vi "nominal teststand convert results.vi"(10 "property bag":refnum<k7>, 11 "Sequence Context In":refnum<k7>) -> (1 "numerics":T1[](array[typedef]), 2 "strings":T2(array[cluster]), 3 "Report Text":string)   [LabVIEW 2020, in "nominal teststand model sequence support.lvlib"]
doc: "Theory of operation:\nFind all AdditionalResults\nGet Parent -> TS -> Start Time\nRecurse down AdditionalResults for data values\n\nParameters.MainSequenceResult->TS.StartTime\nseconds since start of engine for sequence\n\nParameters.MainSequenceResult->TS.SequenceCall.ResultList[0].TS.StartTime\nstep start time <- want this as timestamp for additional results\n\nresults we want\nParameters.MainSequenceResult->TS.SequenceCall.ResultList[0].AdditionalResults[\"result a1\"]"
uses:
  nominal teststand model sequence support.lvlib
  nominal numeric result collection.ctl
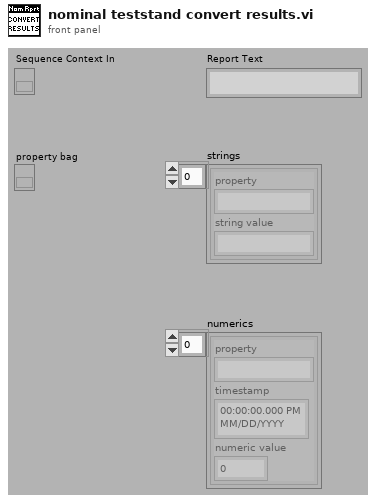
[diagram p1: front panel]
types:
  T1 = typedef "nominal teststand model sequence support.lvlib/nominal numeric result collection.ctl" = cluster{"property":string, "timestamp":timestamp, "numeric value":dbl}
  T2 = cluster{"property":string, "string value":string}[]
  T3 = cluster{timestamp, "strings":cluster{"property":string, "string value":string}[], "numerics":T1[], string}
  T4 = map{string, cluster{"possible timestamp":timestamp, "original property":T1}}
  T5 = map{string, cluster{"possible timestamp":timestamp, "original property":cluster{"property":string, "string value":string}}}
  T6 = cluster{"possible timestamp":timestamp, "original property":cluster{"property":string, "string value":string}}
  T7 = cluster{"possible timestamp":timestamp, "original property":T1}
  T8 = cluster{"property":string, "string value":string}
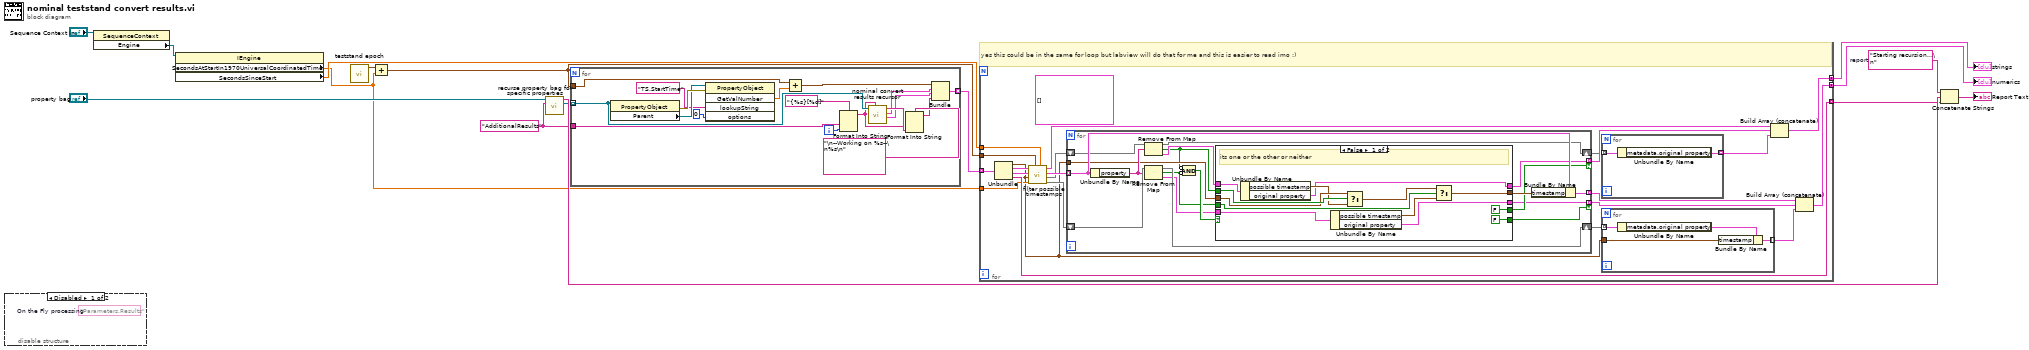
[diagram p0: block diagram]
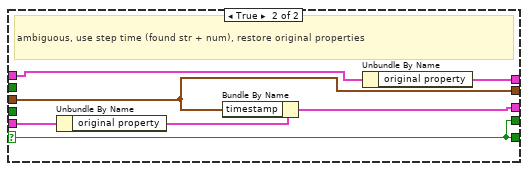
[diagram p2: hidden frame]
diagram:
  w8 = "AdditionalResults" ("search key (match pattern)")
  w15 = "Starting recursion...\n"  # report
  n1 = disable-structure shown="Disabled" {
    frame Disabled {
      (unwired) "Parameters.Results"  # On the Fly processing
    }
    frame Enabled {
    }
  }
  n2 = property class="SequenceContext"(reference="Sequence Context In") -> ("Engine"=w13:refnum<k7>)  [unwired: 1 in, 2 out]
  n3 = property class="IEngine"(reference=w13) -> ("SecondsAtStartIn1970UniversalCoordinatedTime"=w3:dbl, "SecondsSinceStart"=w4:dbl)  [unwired: 1 in, 2 out]
  n4 = call "teststand epoch.vi"() -> ("time stamp"=w12:timestamp)  [unwired: 11 in]
  n5 = Add(x=w12, y=w3) -> (x+y=w5:timestamp)
  n6 = call "recurse property bag for specific properties.vi"("search key (match pattern)"=w8, "property bag"="property bag") -> ("matching properties"=w9:refnum<k7>[], "Report Text"=w10:string)  [unwired: 8 in]
  n7 = for {
    tunnel: w9 -> [w28] mode=indexing
    tunnel: w5 -> [w29]
    tunnel: w8 -> [w24]
    tunnel: [w18] -> w7 mode=indexing
    i -> [w23]
    n8 = property class="PropertyObject"(reference=w28) -> (error out=w33:errorcluster, "Parent"=w32:refnum<k7>)  [unwired: 1 in, 1 out]
    n9 = invoke class="PropertyObject" method="GetValNumber"(reference=w32, error in=w33, "lookupString"="TS.StartTime" ("Lookup String"), "options"=0) -> ("GetValNumber"=w30:dbl)  [unwired: 1 in, 4 out]
    n10 = Add(x=w29, y=w30) -> (x+y=w21:timestamp)
    n11 = Format Into String(format string="{%s}[%d]", w24, w23) -> (resulting string=w22:string)  [unwired: 2 in, 1 out]
    n12 = call "nominal convert results recursor.vi"("hierarchy path"=w22, "property bag"=w28) -> ("numerics"=w19:T1[], "strings"=w20:T2, "Report Text"=w26:string)  [unwired: 7 in]
    n13 = Format Into String(format string="\n--Working on %s--\n%s\n", w22, w26) -> (resulting string=w17:string)  [unwired: 2 in, 1 out]
    n14 = Bundle(w21, "strings"=w20, "numerics"=w19, w17) -> (w18:T3)  [unwired: 1 in]
  }
  n15 = for {
    tunnel: w7 -> [w55] mode=indexing
    tunnel: [w54] -> w6 mode=indexing
    tunnel: w5 -> [w51]
    tunnel: w4 -> [w50]
    tunnel: w3 -> [w49]
    tunnel: [w47] -> w2 mode=concatenating
    tunnel: [w40] -> w1 mode=concatenating
    (unwired) T1[] [] ("numerics")
    # "yes this could be in the same for loop but labview will do that for me and this is easier to read imo :)"
    n16 = Unbundle(w55) -> (w35:timestamp, "strings"=w52:T2, "numerics"=w53:T1[], w54:string)
    n17 = call "filter possible timestamps.vi"("SecondsSinceStart"=w50, "engine start"=w51, "seconds at start"=w49, "step time"=w35, "numerics"=w53, "strings"=w52) -> ("possible timestamp numeric matches"=w44:T4, "possible timestamp string matches"=w45:T5, "remaining numerics"=w46:T1[], "remaining strings"=w48:T2)  [unwired: 2 in]
    n18 = for {
      tunnel: w46 -> [w78] mode=indexing
      tunnel: w35 -> [w68]
      tunnel: [w79] -> w43 mode=indexing
      shift-right: [w74] -> w39
      shift-left: w45 -> [w77]
      shift-right: [w73] -> w37
      shift-left: w44 -> [w76]
      tunnel: [w67] -> w41 mode=indexing if=w66
      tunnel: [w65] -> w42 mode=indexing if=w64
      n19 = Unbundle By Name(w78) -> ("property"=w75:string)
      n20 = Remove From Map(10:w75, 11:w77) -> (1:w70:T6, 2:w63:bool, 3:w74:T5)
      n21 = Remove From Map(10:w75, 11:w76) -> (1:w71:T7, 2:w62:bool, 3:w73:T4)
      n22 = Compound Arithmetic op=AND(invert w63, invert w62) -> (w72:bool)
      n23 = case shown="False" w72 {
        selector: w72 -> [_ w93]
        tunnel: w71 -> [w92 w97]
        tunnel: w70 -> [w91 w99]
        tunnel: [w84 w95] -> w69
        tunnel: w68 -> [w89 w95]
        tunnel: [w80 w98] -> w67
        tunnel: [FALSE w93] -> w66
        tunnel: [w81 w94] -> w65
        tunnel: [FALSE w93] -> w64
        tunnel: w63 -> [w90 _]
        tunnel: w62 -> [w86 _]
        frame False {
          # "its one or the other or neither"
          n24 = Unbundle By Name(w91) -> ("possible timestamp"=w88:timestamp, "original property"=w80:T8)
          n25 = Unbundle By Name(w92) -> ("possible timestamp"=w85:timestamp, "original property"=w81:T1)
          n26 = Select(t=w89, s=w90, f=w88) -> (s? t:f=w87:timestamp)
          n27 = Select(t=w87, s=w86, f=w85) -> (s? t:f=w84:timestamp)
        }
        frame True {
          # "ambiguous, use step time (found str + num), restore original properties"
          n28 = Unbundle By Name(w97) -> ("original property"=w96:T1)
          n29 = Bundle By Name(cluster=w96, "timestamp"=w95) -> (w94:T1)
          n30 = Unbundle By Name(w99) -> ("original property"=w98:T8)
        }
      }
      n31 = Bundle By Name(cluster=w78, "timestamp"=w69) -> (w79:T1)
    }
    n32 = for {
      tunnel: w39 -> [w61] mode=indexing
      tunnel: [w60] -> w38 mode=indexing
      n33 = Unbundle By Name(w61) -> ("metadata.original property"=w60:T8)
    }
    n34 = for {
      tunnel: w37 -> [w59] mode=indexing
      tunnel: [w57] -> w36 mode=indexing
      tunnel: w35 -> [w56]
      n35 = Unbundle By Name(w59) -> ("metadata.original property"=w58:T1)
      n36 = Bundle By Name(cluster=w58, "timestamp"=w56) -> (w57:T1)
    }
    n37 = Build Array (concatenate)(w48, w41, w38) -> (w47:T2)
    n38 = Build Array (concatenate)(w43, w42, w36) -> (w40:T1[])
  }
  "strings" <- w2
  "numerics" <- w1
  n39 = Concatenate Strings(w15, w10, w6) -> (→"Report Text":string)
